vi "[ce] Links to VIs used in FuncVIs.vi"() -> ()   [LabVIEW 2021]
doc: "### DEPRECATED ###\n\nIf you create a stand-alone application that should call FuncVIs, you have two approaches to build it. On the one hand, you can include required FuncVIs to a main application file (dll or exe). On the other hand, you can place FuncVIs libraries separately of the main application file. The second way provides your application with more flexibility because it allows changing and extending a set of FuncVIs without changing other application files. This VI is intended to simplificate creation of such stand-alone applications.\n\nThe FuncVIs are dynamically called VIs; they are not present in hierarchy of any VIs. On this reason, if you build an application without including FuncVIs to the built project, LabVIEW cannot automatically include all required SubVIs to the application. Therefore, some FuncVIs will not be executable because some of their SubVIs are not found.\n\nThis VI contains links to general CalcExpress VIs that are used in FuncVIs. If you include this VI to your building project, it guarantees that all general SubVIs and TypeDefs will be included to stand-alone applications.\n\nImportant Remarks.\n==================\n1. Some FuncVI libraries contain additional VIs that are used by FuncVIs stored in these libraries. This VI does not have links to such VIs.\n2. If any FuncVIs use external VIs in relation to CalcExpress (e.g. LabVIEW Analysis VIs, etc.) you should explicitly include them to your project. \n3. FuncVI search paths are defined in an \"Func - FuncVI search paths.vi\", you should correctly define these paths at either development time or runtime.\n\n::: CalcExpress Toolkit :::\nCopyright (c) 2000-2026 Konstantin Shifershteyn. All rights reserved."
uses:
  cetypes.llb/VarMan Variable Context Handle.ctl
  cetypes.llb/CalcExpress Data Type.ctl
  cetypes.llb/CalcExpress Instance RefNum.ctl
  cetypes.llb/CalcExpress Function Argument Info.ctl
  cetypes.llb/VarMan Error Code.ctl
  cse.llb/CSE Instance RefNum.ctl
panel:
  in  "CSE RefNum":T1
  in  "False":bool
  in  "VarMan error":T2 items=["No error", "Invalid variable type", "Variable not found", "Variable already exists", "Invalid context handle", "Input error", "Invalid data format", "No history attached", "History already attached", "Invalid history parameters", "Wrong variable name", "Wrong alias name", "Non-unique alias", "Alias not found", "No alias associated", "Alias already associated", "Wrong context name", "Non-unique context name", "Context name not found", "Invalid parameter", "Generic error", "Memory Full", "Unrecognized LV error", "Unknown error code"]
  in  "opd info":T3
  in  "CE InstanceRef":T4
  out "error out":bool
  in  "data type":T5=enum."DBL Number"
  in  "VC Handle":T6=-1
  in  "error in":bool
  # "Description of this VI contains comments on building\nstand-alone applications that use CalExpress."
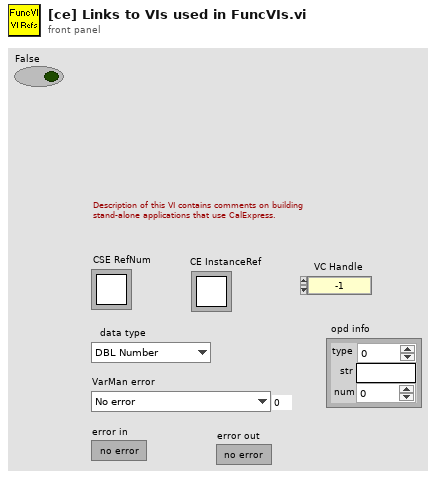
[diagram p1: front panel]
types:
  T1 = typedef "CSE Instance RefNum.ctl" = refnum<k1>
  T2 = typedef "VarMan Error Code.ctl" = u16
  T3 = typedef "CalcExpress Function Argument Info.ctl" = cluster{"type":u32, "str":string, "num":dbl}
  T4 = typedef "CalcExpress Instance RefNum.ctl" = refnum<k1>
  T5 = typedef "CalcExpress Data Type.ctl" = enum32{"String", "DBL Number", "identifier", "1D Array of DBL", "2D Array of DBL", "CDB Number", "1D Array of CDB", "2D Array of CDB", "1D Array of String", "2D Array of String", "Unknown data type"}
  T6 = typedef "VarMan Variable Context Handle.ctl" = i32
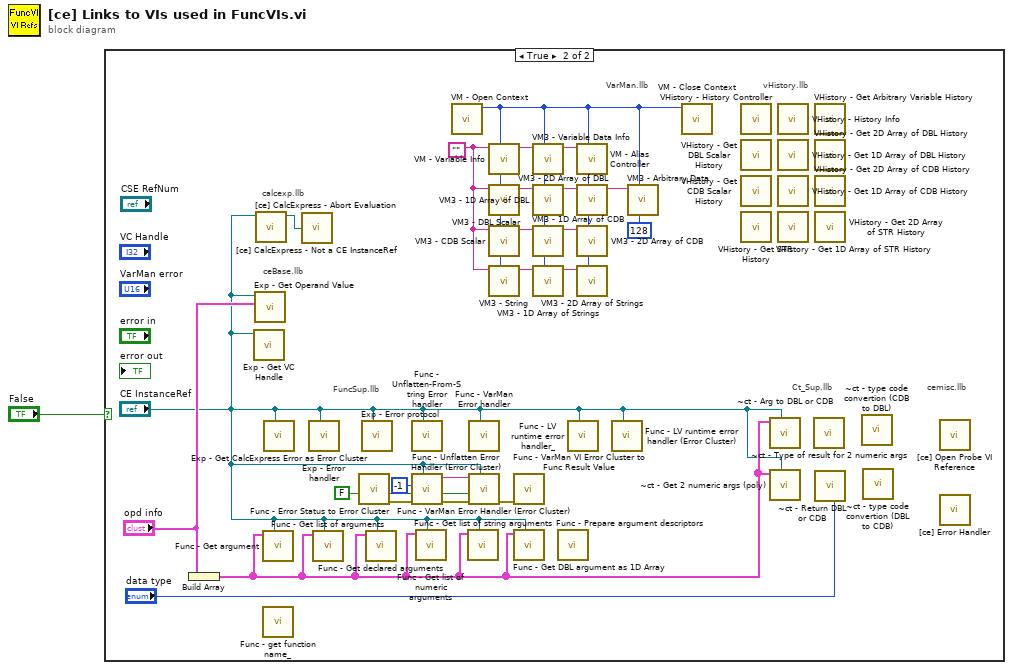
[diagram p0: block diagram]
diagram:
  n1 = case shown="True" "False" {
    frame False {
    }
    frame True {
      w8 = ""
      # "calcexp.llb"
      # "vHistory.llb"
      # "VarMan.llb"
      # "cemisc.llb"
      # "ceBase.llb"
      # "Ct_Sup.llb"
      # "FuncSup.llb"
      n2 = Build Array("opd info") -> (w24:T3[])
      n3 = call "Exp - Get VC Handle.vi"("InstanceRef"="CE InstanceRef") -> ()  [unwired: 5 in, 4 out]
      n4 = call "Exp - Get Operand Value.vi"("op info"="opd info", "InstanceRef"="CE InstanceRef") -> ()  [unwired: 4 in, 4 out]
      n5 = call "[ce] CalcExpress - Abort Evaluation.vi"("CE InstanceRef"="CE InstanceRef") -> ("dup CE InstanceRef"=w23:T4)  [unwired: 7 in, 1 out]
      n6 = call "Func - Get argument.vi"("InstanceRef"="CE InstanceRef", "arg list"=w24) -> ()  [unwired: 4 in, 4 out]
      n7 = call "Func - get function name_.vi"() -> ()  [unwired: 9 in, 3 out]
      n8 = call "Exp - Get CalcExpress Error as Error Cluster.vi"("InstanceRef"="CE InstanceRef") -> ()  [unwired: 9 in, 2 out]
      n9 = call "[ce] CalcExpress - Not a CE InstanceRef.vi"("CE InstanceRef"=w23) -> ()  [unwired: 2 out]
      n10 = call "Exp - Error handler.vi"("InstanceRef"="CE InstanceRef") -> ()  [unwired: 8 in, 3 out]
      n11 = call "Func - Get list of arguments.vi"("InstanceRef"="CE InstanceRef", "arg list"=w24) -> ()  [unwired: 6 in, 4 out]
      n12 = call "Func - Error Status to Error Cluster.vi"("error status in"=FALSE) -> ("Error Cluster out"=w22:errorcluster, "error status out"=w17:bool)  [unwired: 9 in]
      n13 = call "Exp - Error protocol.vi"("InstanceRef"="CE InstanceRef") -> ()  [unwired: 7 in, 2 out]
      n14 = call "Func - Get declared arguments.vi"("InstanceRef"="CE InstanceRef", "arg list"=w24) -> ()  [unwired: 6 in, 4 out]
      n15 = call "Func - Unflatten-From-String Error handler.vi"("InstanceRef"="CE InstanceRef") -> ()  [unwired: 8 in, 1 out]
      n16 = call "Func - Unflatten Error Handler (Error Cluster).vi"("InstanceRef"="CE InstanceRef", "Unflatten Error Cluster"=w22, "error status before"=w17, "argument number"=-1) -> ("Error Cluster out"=w21:errorcluster, "error status out"=w18:bool, "dup name"=w19:string)  [unwired: 5 in]
      n17 = call "Func - Get list of numeric arguments.vi"("InstanceRef"="CE InstanceRef", "arg list"=w24) -> ()  [unwired: 6 in, 2 out]
      n18 = call "VM - Open Context.vi"() -> ("VC Handle out"=w2:T6)  [unwired: 9 in, 2 out]
      n19 = call "Func - Get list of string arguments.vi"("InstanceRef"="CE InstanceRef", "arg list"=w24) -> ()  [unwired: 6 in, 2 out]
      n20 = call "Func - VarMan Error handler.vi"("InstanceRef"="CE InstanceRef") -> ()  [unwired: 6 in, 3 out]
      n21 = call "Func - VarMan Error Handler (Error Cluster).vi"("InstanceRef"="CE InstanceRef", "VarMan VI error in"=w21, "error status before"=w18, "var name"=w19) -> ("error out"=w20:errorcluster)  [unwired: 5 in, 2 out]
      n22 = call "VM - Variable Info.vi"("VC Handle"=w2, "name_spec"=w8) -> ("var name"=w13:string)  [unwired: 4 in, 5 out]
      n23 = call "VM3 - DBL Scalar.vi"("VC Handle"=w2, "name_spec"=w8) -> ("dup name_spec"=w11:string)  [unwired: 6 in, 3 out]
      n24 = call "VM3 - CDB Scalar.vi"("VC Handle"=w2, "name_spec"=w8) -> ("dup name_spec"=w7:string)  [unwired: 6 in, 3 out]
      n25 = call "VM3 - String.vi"("VC Handle"=w2, "name_spec"=w8) -> ("dup name_spec"=w5:string)  [unwired: 6 in, 3 out]
      n26 = call "Func - VarMan VI Error Cluster to Func Result Value.vi"("VarMan VI error in"=w20) -> ()  [unwired: 10 in, 1 out]
      n27 = call "Func - Get DBL argument as 1D Array.vi"("InstanceRef"="CE InstanceRef", "arg list"=w24) -> ()  [unwired: 6 in, 4 out]
      n28 = call "VM3 - Variable Data Info.vi"("VC Handle"=w2, "name_spec"=w13) -> ("dup name_spec"=w12:string)  [unwired: 4 in, 5 out]
      n29 = call "VM3 - 1D Array of DBL.vi"("VC Handle"=w2, "name_spec"=w11) -> ("dup name_spec"=w10:string)  [unwired: 6 in, 3 out]
      n30 = call "VM3 - 1D Array of CDB.vi"("VC Handle"=w2, "name_spec"=w7) -> ("dup name_spec"=w6:string)  [unwired: 6 in, 3 out]
      n31 = call "VM3 - 1D Array of Strings.vi"("VC Handle"=w2, "name_spec"=w5) -> ("dup name_spec"=w4:string)  [unwired: 6 in, 3 out]
      n32 = call "Func - Prepare argument descriptors.vi"() -> ()  [unwired: 8 in, 2 out]
      n33 = call "Func - LV runtime error handler_.vi"("InstanceRef"="CE InstanceRef") -> ()  [unwired: 10 in, 1 out]
      n34 = call "VM - Alias Controller.vi"("VC Handle"=w2, "name_spec"=w12) -> ()  [unwired: 6 in, 4 out]
      n35 = call "VM3 - 2D Array of DBL.vi"("VC Handle"=w2, "name_spec"=w10) -> ("dup name_spec"=w9:string)  [unwired: 6 in, 3 out]
      n36 = call "VM3 - 2D Array of CDB.vi"("VC Handle"=w2, "name_spec"=w6) -> ()  [unwired: 6 in, 4 out]
      n37 = call "VM3 - 2D Array of Strings.vi"("VC Handle"=w2, "name_spec"=w4) -> ()  [unwired: 6 in, 4 out]
      n38 = call "Func - LV runtime error handler (Error Cluster).vi"("InstanceRef"="CE InstanceRef") -> ()  [unwired: 5 in, 4 out]
      n39 = call "VM3 - Arbitrary Data.vi"("var type in"=u32 128 ("var type"), "VC Handle"=w2, "name_spec"=w9) -> ()  [unwired: 4 in, 5 out]
      n40 = call "VM - Close Context.vi"("VC Handle"=w2) -> ()  [unwired: 9 in, 2 out]
      n41 = call "VHistory - History Controller.vi"() -> ()  [unwired: 8 in, 4 out]
      n42 = call "VHistory - Get DBL Scalar History.vi"() -> ()  [unwired: 7 in, 5 out]
      n43 = call "VHistory - Get CDB Scalar History.vi"() -> ()  [unwired: 7 in, 5 out]
      n44 = call "VHistory - Get STR History.vi"() -> ()  [unwired: 7 in, 5 out]
      n45 = call "~ct - Arg to DBL or CDB.vi"("InstanceRef"="CE InstanceRef", "args list"=w24) -> ()  [unwired: 3 in, 7 out]
      n46 = call "~ct - Get 2 numeric args (poly).vi"("InstanceRef"="CE InstanceRef", "args list"=w24) -> ()  [unwired: 4 in, 6 out]
      n47 = call "VHistory - History Info.vi"() -> ()  [unwired: 7 in, 5 out]
      n48 = call "VHistory - Get 1D Array of DBL History.vi"() -> ()  [unwired: 7 in, 5 out]
      n49 = call "VHistory - Get 1D Array of CDB History.vi"() -> ()  [unwired: 7 in, 5 out]
      n50 = call "VHistory - Get 1D Array of STR History.vi"() -> ()  [unwired: 7 in, 5 out]
      n51 = call "~ct - Type of result for 2 numeric args.vi"() -> ()  [unwired: 7 in, 3 out]
      n52 = call "VHistory - Get Arbitrary Variable History.vi"() -> ()  [unwired: 7 in, 5 out]
      n53 = call "VHistory - Get 2D Array of DBL History.vi"() -> ()  [unwired: 7 in, 5 out]
      n54 = call "VHistory - Get 2D Array of CDB History.vi"() -> ()  [unwired: 7 in, 5 out]
      n55 = call "VHistory - Get 2D Array of STR History.vi"() -> ()  [unwired: 7 in, 5 out]
      n56 = call "~ct - Return DBL or CDB.vi"("type"="data type") -> ()  [unwired: 9 in, 2 out]
      n57 = call "~ct - type code convertion (CDB to DBL).vi"() -> ()  [unwired: 5 in, 1 out]
      n58 = call "~ct - type code convertion (DBL to CDB).vi"() -> ()  [unwired: 5 in, 1 out]
      n59 = call "[ce] Open Probe VI Reference.vi"() -> ()  [unwired: 9 in, 3 out]
      n60 = call "[ce] Error Handler.vi"() -> ()  [unwired: 10 in, 2 out]
    }
  }
